vi "Cmd HO (TT).vi"(8 "error in (no error)":errorcluster caption="에러 입력(에러 없음)", 11 "CO3000 입력":refnum<class "CO3000.lvclass">) -> (0 "error out":errorcluster caption="에러 출력", 3 "CO3000 출력":refnum<class "CO3000.lvclass">)   [LabVIEW 2023, in "Turn Table and Mast.lvlib" / "CO3000.lvclass"]
uses:
  CO3000.lvclass
  CO3000.lvclass/CO3000.ctl
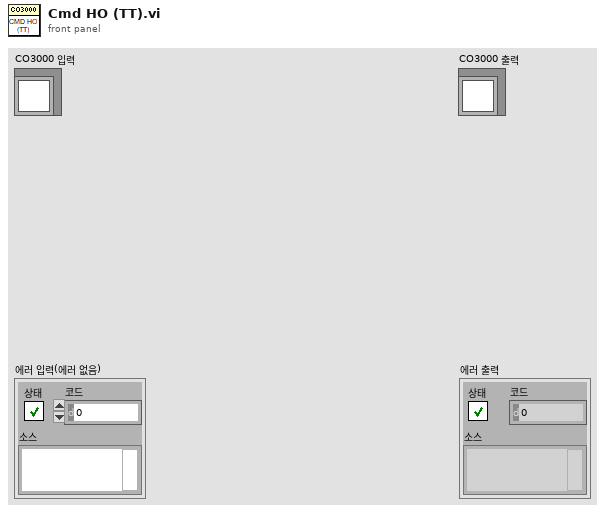
[diagram p1: front panel]
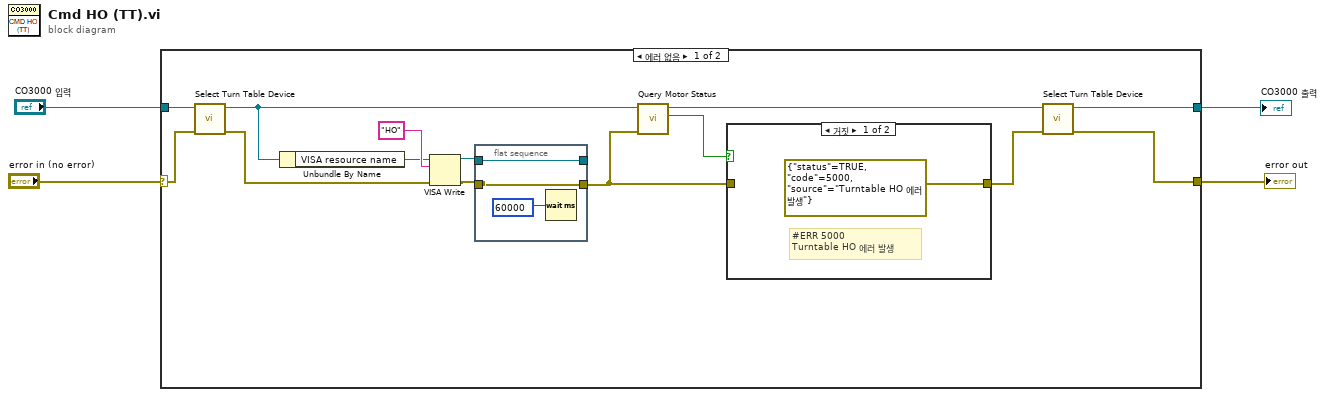
[diagram p0: block diagram]
diagram:
  n1 = case shown="에러 없음" "error in (no error)" {
    selector: "error in (no error)" -> [w5 w25]
    tunnel: [w6 w25] -> w1
    tunnel: [w15 w24] -> w3
    tunnel: "CO3000 입력" -> [w13 w24]
    frame No Error {
      n2 = call "Select Turn Table Device.vi"("error in (no error)"=w5, "CO3000 in"=w13) -> ("error out"=w9:errorcluster, "CO3000 out"=w11:refnum<class "CO3000.lvclass">)  [unwired: 8 in]
      n3 = Unbundle By Name(w11) -> ("VISA resource name"=w10:refnum<visa-resource-name>)
      n4 = VISA Write(VISA resource name=w10, write buffer="HO" ("버퍼 쓰기"), error in (no error)=w9) -> (VISA resource name out=w17:refnum<visa-resource-name>, error out=w16:errorcluster)  [unwired: 1 out]
      n5 = flat-sequence {
        tunnel: w16 -> [w22]
        tunnel: w17 -> [w21]
        tunnel: [w22] -> w8
        tunnel: [w21] -> _
        frame #0 {
          n6 = Wait (ms)(milliseconds to wait=u32 60000 ("대기 시간 (ms)")) -> ()  [unwired: 1 out]
        }
      }
      n7 = call-dynamic "Query Motor Status.vi"("error in (no error)"=w8, "CO3000 in"=w11) -> ("Motor Stop?"=w12:bool, "CO3000 out"=w14:refnum<class "CO3000.lvclass">)  [unwired: 7 in, 1 out]
      n8 = case shown="거짓" w12 {
        tunnel: [errorcluster {"status"=TRUE, "code"=5000, "source"="Turntable HO 에러 발생"} ("에러 상수") w20] -> w7
        tunnel: w8 -> [_ w20]
        frame False {
          # "#ERR 5000\nTurntable HO 에러 발생"
        }
        frame True {
        }
      }
      n9 = call "Select Turn Table Device.vi"("error in (no error)"=w7, "CO3000 in"=w14) -> ("error out"=w6:errorcluster, "CO3000 out"=w15:refnum<class "CO3000.lvclass">)  [unwired: 8 in]
    }
    frame Error {
    }
  }
  "error out" <- w1
  "CO3000 출력" <- w3
